vi "A Version Explorer - UI.vi"() -> ()   [LabVIEW 2020, in "A Version Explorer.lvlib"]
uses:
  A Version Explorer.lvlib
  Session/Session.lvclass
  <vilib>/Utility/miscctls.llb/LVRowAndColumnUnsignedTypeDef.ctl
  <vilib>/Utility/miscctls.llb/LVRowAndColumnTypeDef.ctl
  Session/Session.lvclass/Session.ctl
  <userlib>/_OpenG.lib/file/file.llb/Valid Path - Traditional__ogtk.vi
  <userlib>/_OpenG.lib/array/array.llb/Index 1D Array Elements (String)__ogtk.vi
panel:
  in  "Project Folder":path
  in  "Select All/Some/None":enum8{"False", "True", "Mixed"}(c332)
  in  "Refresh":bool
  in  "Save for Previous Version":bool
  in  "LabVIEW Version":string(combo)
  in  "Files":i32[](listbox)
  out "Status":string
  in  "OK":bool
  # "1) Select a Project Folder with files you wish to save to an earlier version of LabVIEW.\n    (Make note of the current LabVIEW version of each file using the listbox below.)"
  # "2) Select the project files in the listbox below that you\nwish to save to a different LabVIEW Version.\n\n(Ctrl+A selects all files, Ctrl+Click selects individual files.)"
  # "3) Select the target LabVIEW version.\n4) Press \"Save Selected Files\""
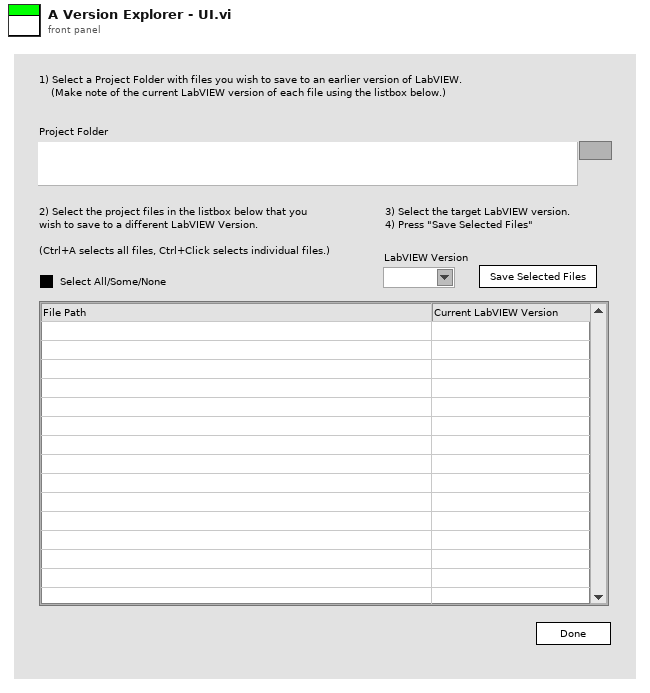
[diagram p1: front panel]
types:
  T1 = enum32{"Invalid", "Standard", "Closed", "Hidden", "Minimized", "Maximized"}
  T2 = enum32{"invalid app kind", "Development System", "Run Time System", "Student Edition", "Embedded LabVIEW", "Evaluation", "Custom"}
  T3 = typedef "LVRowAndColumnUnsignedTypeDef.ctl" = cluster{"Row":u32, "Column":u32}
  T4 = typedef "LVRowAndColumnTypeDef.ctl" = cluster{"Row":i32, "Column":i32}
  T5 = typedef "eventvkey.ctl" = enum16{"ASCII", "Enter", "Return", "Shift", "Ctrl", "Alt", "Cmd", "Opt", "Caps", "NumLock", "Clear", "Break", "Up", "Down", "Left", "Right", "Insert", "Delete", "Home", "End", "PageUp", "PageDown", "Escape", "Help", "Pause", "ScrollLock", "F1", "F2", "F3", "F4", "F5", "F6", "F7", "F8", "F9", "F10", "F11", "F12", "F13", "F14", "F15", "F16", "F17", "F18", "F19", "F20", "F21", "F22", "F23", "F24", "Play", "VolumeUp", "VolumeDown", "Mute", "Two Byte Char"}
  T6 = cluster{"Shift":bool, "Ctrl":bool, "Alt":bool, "Cmd":bool, "Opt":bool}
  T7 = cluster{"Core":cluster{"Current VI Reference":refnum<vi>, "Close Panel on Exit?":bool}, "Your Boolean data":bool, "Session":refnum<class "Session.lvclass">}
  T8 = cluster{"Current VI Reference":refnum<vi>, "Close Panel on Exit?":bool}
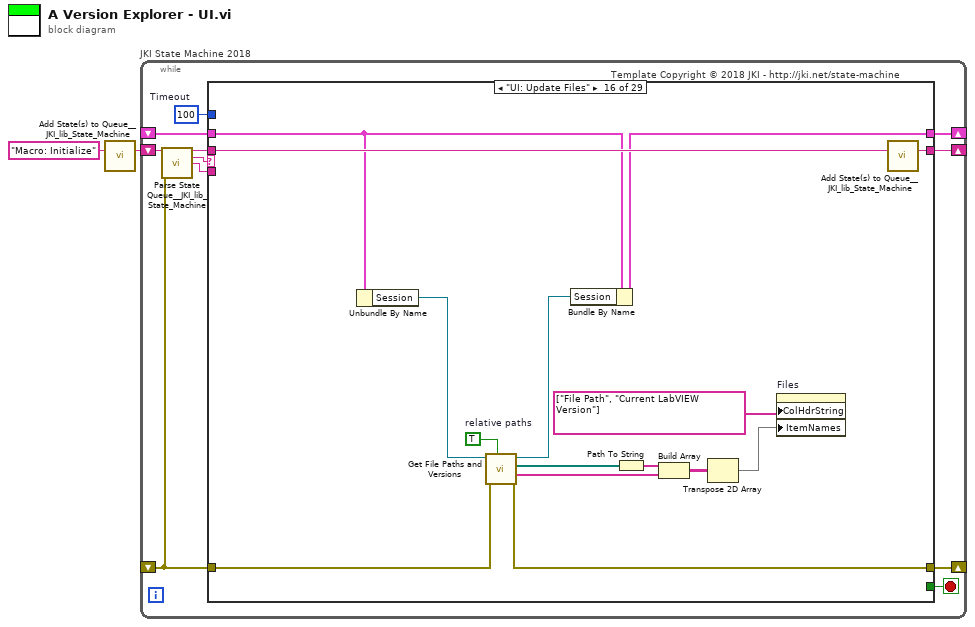
[diagram p0: block diagram]
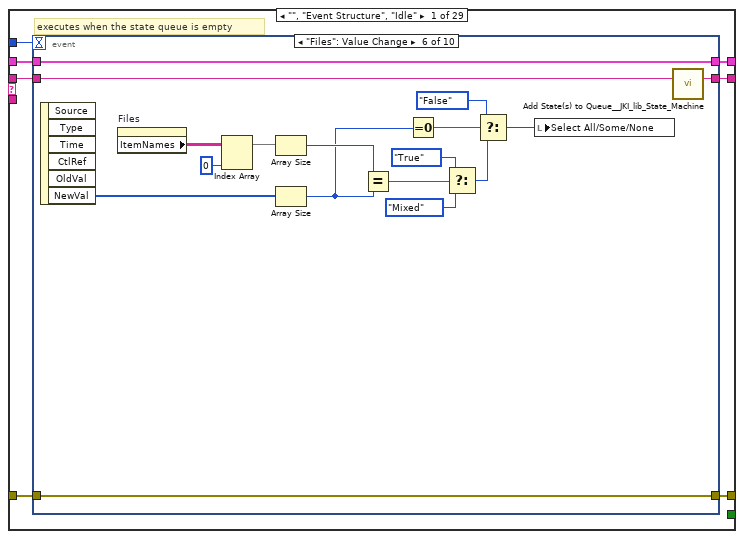
[diagram p2: hidden frame]
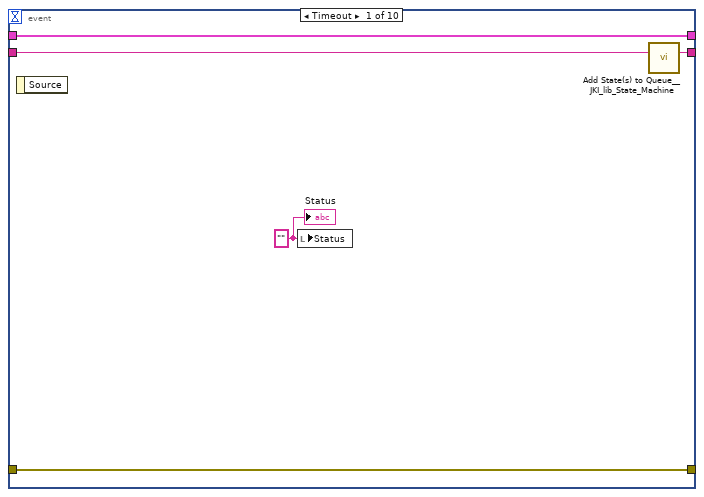
[diagram p3: hidden frame]
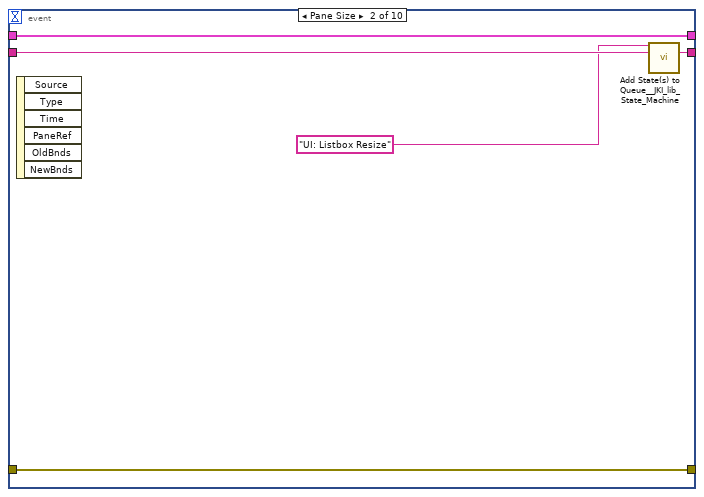
[diagram p4: hidden frame]
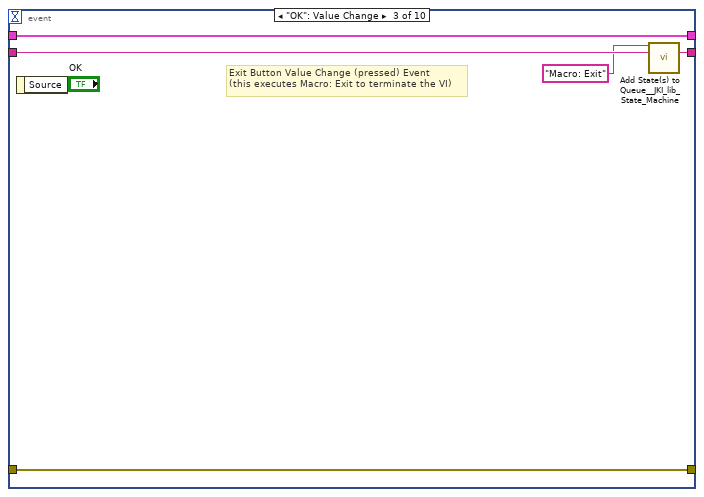
[diagram p5: hidden frame]
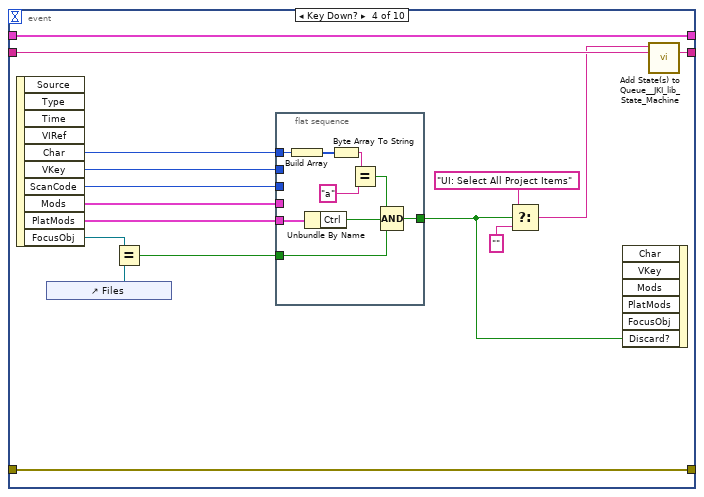
[diagram p6: hidden frame]
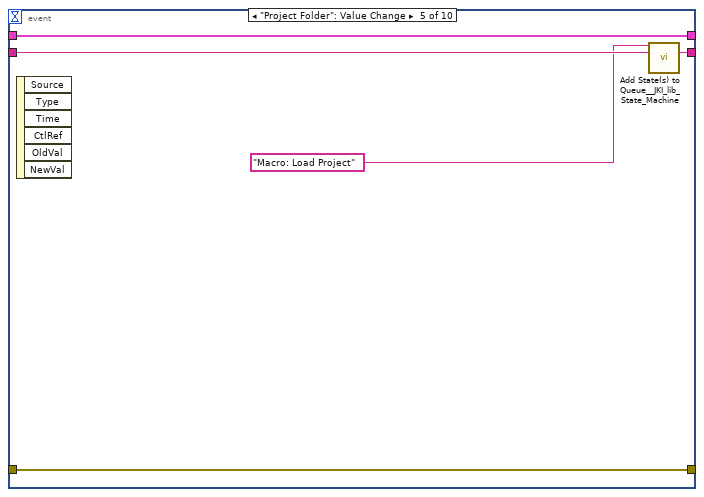
[diagram p7: hidden frame]
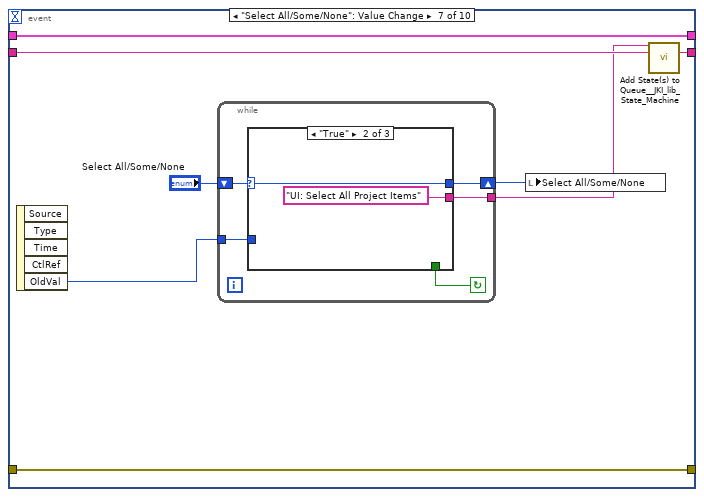
[diagram p8: hidden frame]
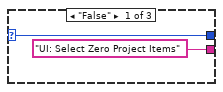
[diagram p9: hidden frame]
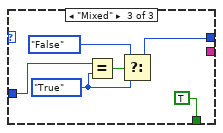
[diagram p10: hidden frame]
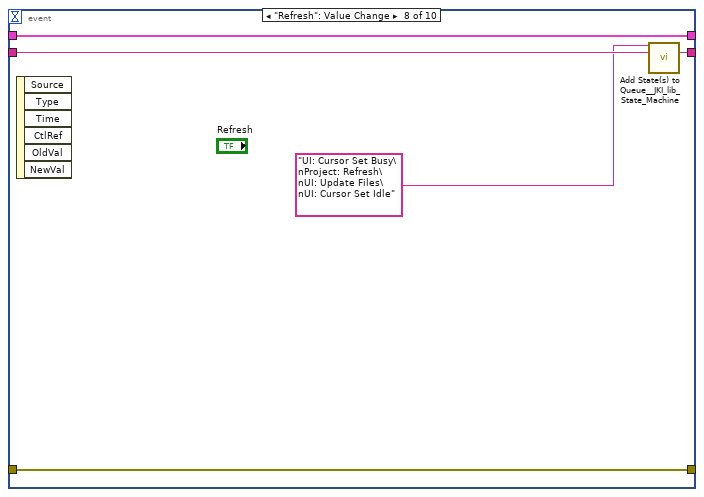
[diagram p11: hidden frame]
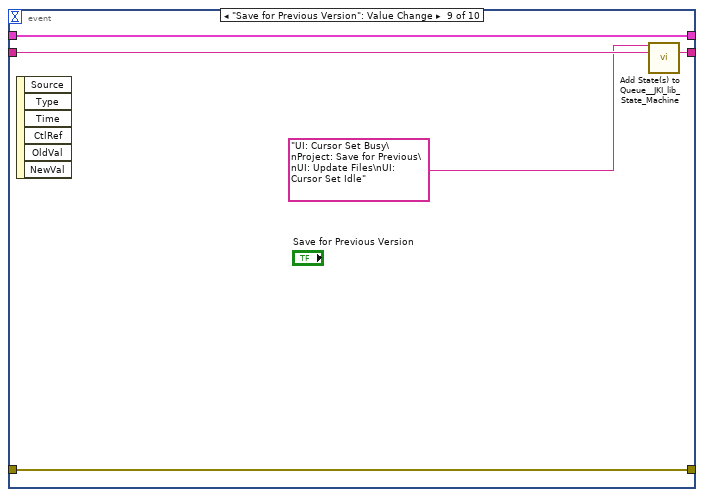
[diagram p12: hidden frame]
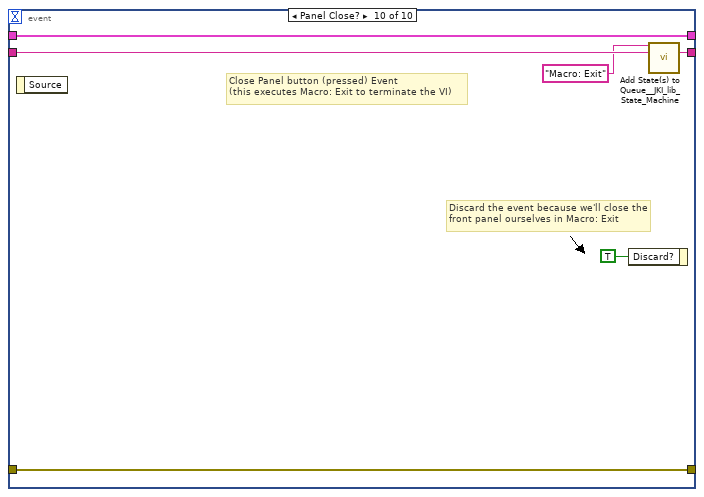
[diagram p13: hidden frame]
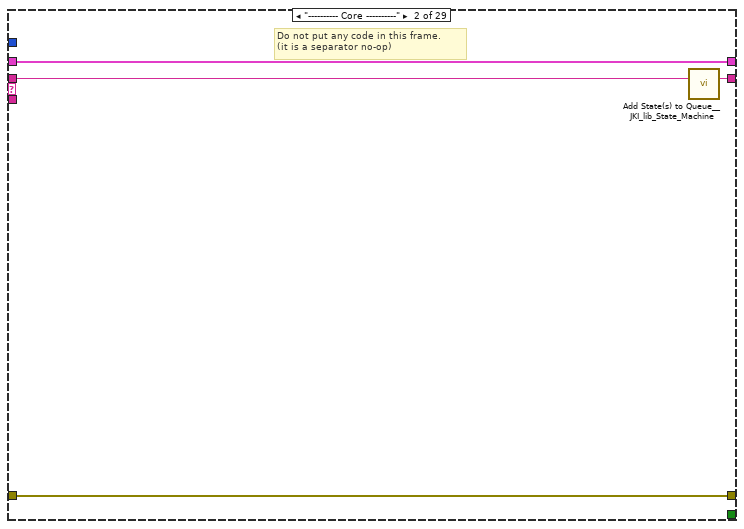
[diagram p14: hidden frame]
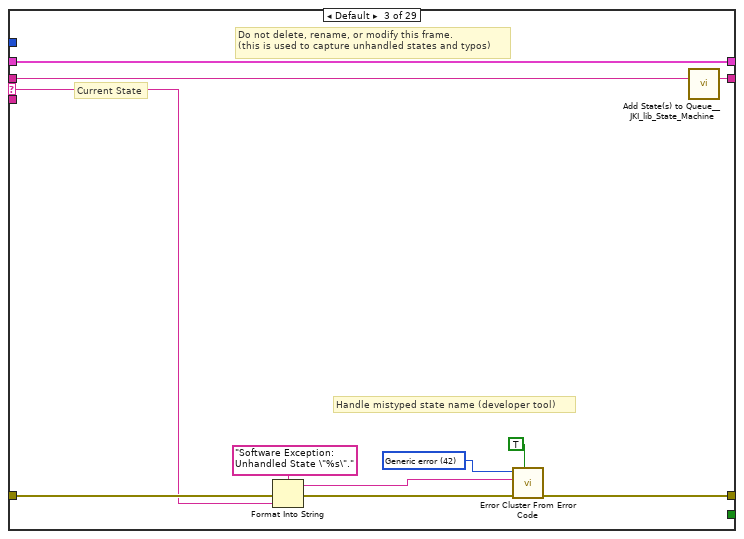
[diagram p15: hidden frame]
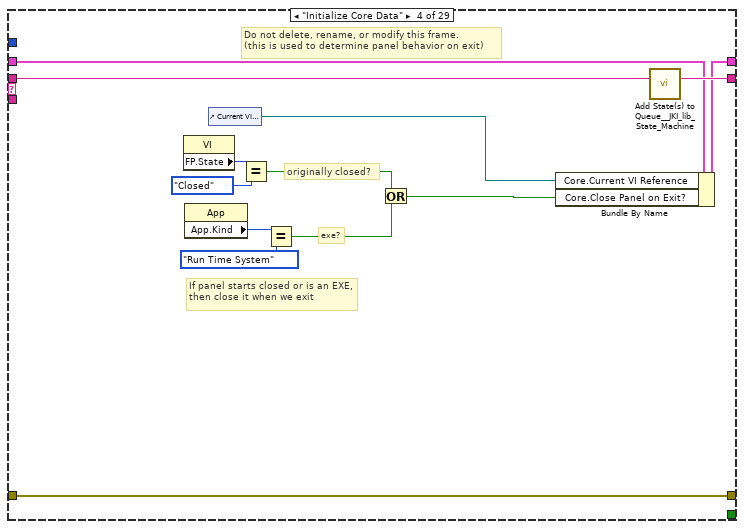
[diagram p16: hidden frame]
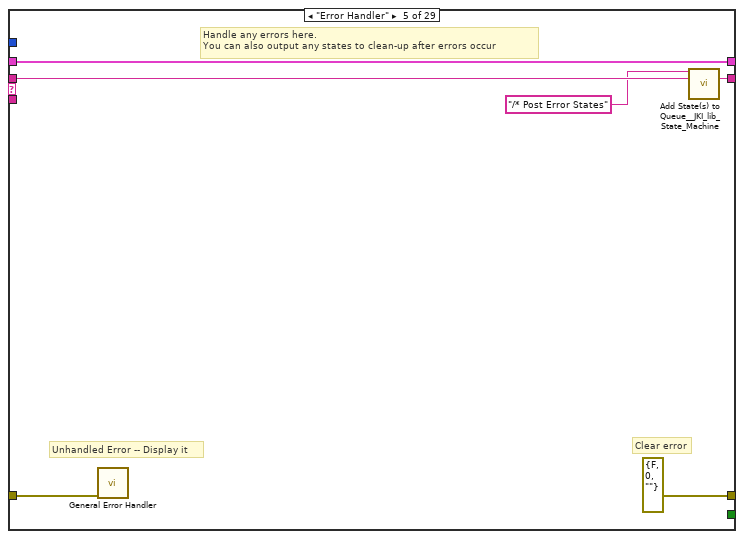
[diagram p17: hidden frame]
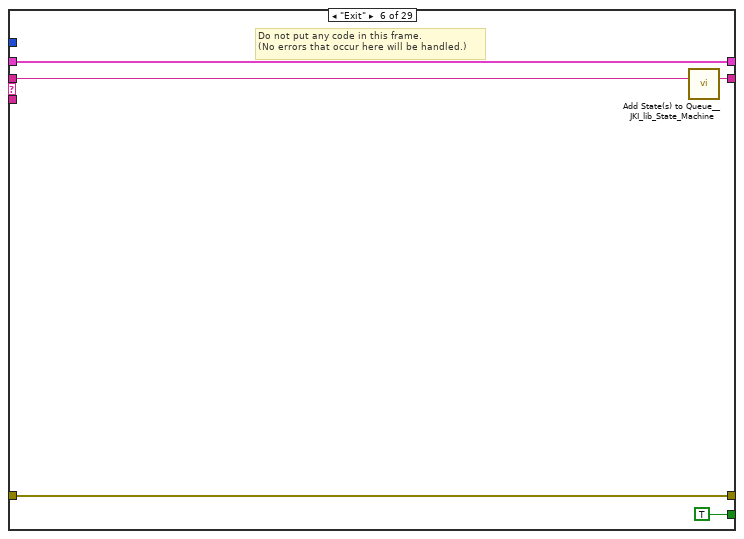
[diagram p18: hidden frame]
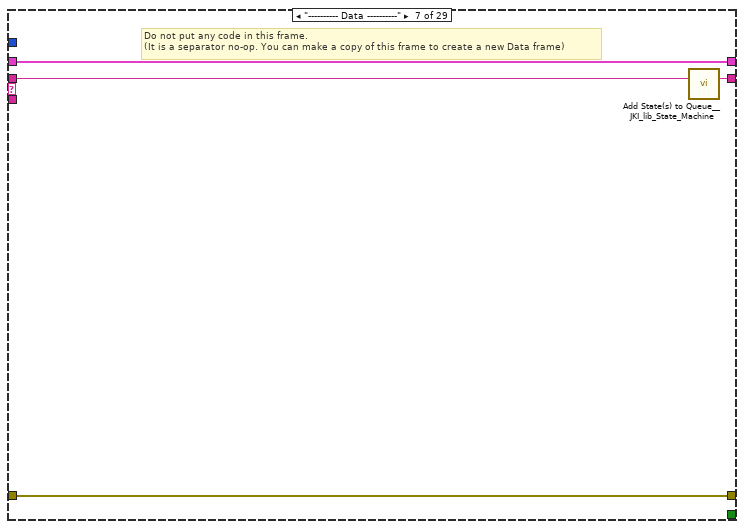
[diagram p19: hidden frame]
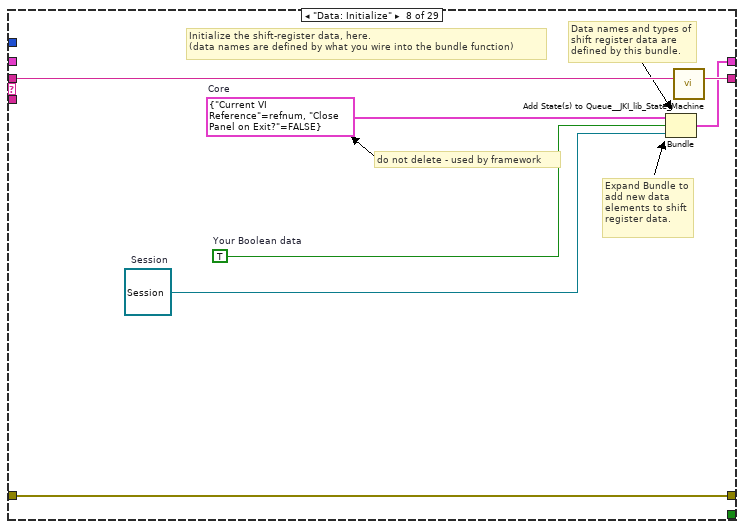
[diagram p20: hidden frame]
diagram:
  n1 = call <vilib>:"Add State(s) to Queue__JKI_lib_State_Machine.vi"("State(s) in (\"\")"="Macro: Initialize") -> ("States Out"=w2:string)  [unwired: 14 in]
  n2 = while "JKI State Machine 2018" {
    shift-right: [w6] -> _
    shift-left: _ -> [w5]
    shift-right: [w9] -> _
    shift-left: _ -> [w3]
    shift-right: [w8] -> _
    shift-left: w2 -> [w10]
    stop <- w7 stop-if-true
    w4 = 100  # Timeout
    # "Template Copyright © 2018 JKI - http://jki.net/state-machine"
    n3 = call <vilib>:"Parse State Queue__JKI_lib_State_Machine.vi"("State Queue"=w10, "Error In (no error)"=w3) -> ("Remaining States"=w12:string, "Current State"=w13:string, "Arguments"=w11:string)  [unwired: 11 in]
    n4 = case shown="\"UI: Update Files\"" w13 {
      selector: w13 -> [_ _ w126 _ _ _ _ _ _ _ _ _ _ _ _ _ _ _ _ _ _ _ _ _ _ _ _ _ _]
      tunnel: w12 -> [w20 w125 w130 w149 w155 w160 w164 w171 w177 w181 w185 w189 w196 w203 w208 w223 w228 w237 w247 w253 w264 w333 w343 w348 w358 w362 w373 w382 w401]
      tunnel: w11 -> [_ _ _ _ _ _ _ _ _ _ _ _ _ _ _ _ _ _ _ w248 w258 _ _ _ _ _ _ _ _]
      tunnel: w5 -> [w18 w122 w128 w142 w152 w158 w161 _ w172 w178 w182 w186 w193 w200 w205 w212 w226 w235 w245 w251 w260 w330 w340 w345 w355 w360 w371 w376 w398]
      tunnel: [w17 w123 w132 w146 errorcluster {"status"=FALSE, "code"=0, "source"=""} ("error out") w157 w162 w168 w173 w179 w183 w187 w194 w201 w206 w215 w225 w234 w244 w249 w261 w331 w341 w346 w356 w359 w367 w378 w399] -> w9
      tunnel: w3 -> [w16 w123 w131 w146 w151 w157 w162 w168 w174 w179 w183 w187 w194 w201 w206 w214 w225 w234 w244 w250 w262 w331 w341 w346 w356 w359 w366 w379 w386]
      tunnel: [w19 w124 w129 w148 w154 w159 w163 w170 w176 w180 w184 w188 w195 w202 w207 w222 w227 w236 w246 w252 w263 w332 w342 w347 w357 w361 w372 w381 w400] -> w8
      tunnel: [_ _ _ _ _ TRUE _ _ _ _ _ _ _ _ _ _ _ _ _ _ _ _ _ _ _ _ _ _ _] -> w7
      tunnel: [w15 w122 w128 w147 w152 w158 w161 w169 w172 w178 w182 w186 w193 w200 w205 w210 w226 w235 w245 w251 w260 w330 w340 w345 w355 w360 w365 w380 w397] -> w6
      tunnel: w4 -> [w14 _ _ _ _ _ _ _ _ _ _ _ _ _ _ _ _ _ _ _ _ _ _ _ _ _ _ _ _]
      frame "", "Event Structure", "Idle" {
        # "executes when the state queue is empty"
        n5 = event shown="[5] \"Files\": Value Change" {
          selector: _ -> [_ _ _ _ _ _ _ _ _ _]
          dyn-events: _ -> [_ _ _ _ _ _ _ _ _ _]
          timeout: w14 -> [_ _ _ _ _ _ _ _ _ _]
          tunnel: w20 -> [w25 w30 w35 w51 w65 w82 w90 w110 w115 w121]
          tunnel: [w24 w29 w34 w50 w64 w81 w89 w109 w114 w120] -> w19
          tunnel: w18 -> [w22 w27 w32 w48 w62 w79 w87 w107 w112 w118]
          tunnel: [w23 w28 w33 w49 w63 w80 w88 w108 w113 w119] -> w17
          tunnel: w16 -> [w23 w28 w33 w49 w63 w80 w88 w108 w113 w119]
          tunnel: [w22 w27 w32 w48 w62 w79 w87 w107 w112 w118] -> w15
          event Timeout {
            w21 = "" ("Status")
            n6 = event-data() -> ()  [unwired: 1 in, 1 out]
            n7 = local write "Status"(w21) -> ()
            n8 = call <vilib>:"Add State(s) to Queue__JKI_lib_State_Machine.vi"("State(s) in (\"\")"=w25) -> ("States Out"=w24:string)  [unwired: 14 in]
            "Status" <- w21
          }
          event Pane Size {
            n9 = event-data() -> ()  [unwired: 1 in, 6 out]
            n10 = call <vilib>:"Add State(s) to Queue__JKI_lib_State_Machine.vi"("State(s) in Front (\"\")"="UI: Listbox Resize" ("Status"), "State(s) in (\"\")"=w30) -> ("States Out"=w29:string)  [unwired: 13 in]
          }
          event "OK": Value Change {
            # "Exit Button Value Change (pressed) Event\n(this executes Macro: Exit to terminate the VI)"
            n11 = event-data() -> ()  [unwired: 1 in, 1 out]
            n12 = call <vilib>:"Add State(s) to Queue__JKI_lib_State_Machine.vi"("State(s) in Front (\"\")"="Macro: Exit", "State(s) in (\"\")"=w35) -> ("States Out"=w34:string)  [unwired: 13 in]
          }
          event Key Down? {
            n13 = event-data() -> ("Char"=w41:i16, "VKey"=w42:T5, "ScanCode"=w43:i16, "Mods"=w47:cluster{"Num Pad":bool, "Menu Key":bool}, "PlatMods"=w46:T6, "FocusObj"=w45:refnum<vi>)  [unwired: 1 in, 4 out]
            n14 = control-ref of="Files"() -> (w44:refnum<vi>)
            n15 = Equal?(x=w45, y=w44) -> (x = y?=w40:bool)
            n16 = flat-sequence {
              tunnel: w47 -> [_]
              tunnel: w46 -> [w60]
              tunnel: w43 -> [_]
              tunnel: w42 -> [_]
              tunnel: w41 -> [w59]
              tunnel: w40 -> [w53]
              tunnel: [w52] -> w39
              frame #0 {
                n17 = Build Array(w59) -> (w58:i16[])
                n18 = Unbundle By Name(w60) -> ("Ctrl"=w54:bool)
                n19 = Byte Array To String(unsigned byte array=w58) -> (string=w57:string)
                n20 = Equal?(x=w57, y="a" ("string")) -> (x = y?=w55:bool)
                n21 = Compound Arithmetic op=AND(w55, w54, w53) -> (w52:bool)
              }
            }
            n22 = Select(t="UI: Select All Project Items", s=w39, f="") -> (s? t:f=w36:string)
            n23 = event-data("Discard?"=w39) -> ()  [unwired: 6 in, 1 out]
            n24 = call <vilib>:"Add State(s) to Queue__JKI_lib_State_Machine.vi"("State(s) in Front (\"\")"=w36, "State(s) in (\"\")"=w51) -> ("States Out"=w50:string)  [unwired: 13 in]
          }
          event "Project Folder": Value Change {
            n25 = event-data() -> ()  [unwired: 1 in, 6 out]
            n26 = call <vilib>:"Add State(s) to Queue__JKI_lib_State_Machine.vi"("State(s) in Front (\"\")"="Macro: Load Project", "State(s) in (\"\")"=w65) -> ("States Out"=w64:string)  [unwired: 13 in]
          }
          event "Files": Value Change {
            n27 = event-data() -> ("NewVal"=w77:i32[])  [unwired: 1 in, 5 out]
            n28 = property on="Files" class="MCListbox (strict)"() -> ("ItemNames"=w78:string[][])  [unwired: 2 in, 2 out]
            n29 = Index Array(array=w78, index (col)=0 ("disabled index (col)")) -> (element=w75:string[])  [unwired: 1 in]
            n30 = Array Size(array=w75) -> (size(s)=w76:i32)
            n31 = Array Size(array=w77) -> (size(s)=w73:i32)
            n32 = Equal?(x=w76, y=w73) -> (x = y?=w69:bool)
            n33 = Equal To 0?(x=w73) -> (x = 0?=w72:bool)
            n34 = Select(t=enum8{"False", "True", "Mixed"}."True" ("Select All/Some/None"), s=w69, f=enum8{"False", "True", "Mixed"}."Mixed" ("Select All/Some/None")) -> (s? t:f=w66:enum8{"False", "True", "Mixed"})
            n35 = Select(t=enum8{"False", "True", "Mixed"}."False" ("Select All/Some/None"), s=w72, f=w66) -> (s? t:f=w70:enum8{"False", "True", "Mixed"})
            n36 = local write "Select All/Some/None"(w70) -> ()
            n37 = call <vilib>:"Add State(s) to Queue__JKI_lib_State_Machine.vi"("State(s) in (\"\")"=w82) -> ("States Out"=w81:string)  [unwired: 14 in]
          }
          event "Select All/Some/None": Value Change {
            n38 = event-data() -> ("OldVal"=w84:enum8{"False", "True", "Mixed"})  [unwired: 1 in, 4 out]
            n39 = while {
              tunnel: [w94] -> w85
              tunnel: w84 -> [w93]
              shift-right: [w91] -> w83
              shift-left: "Select All/Some/None" -> [w95]
              stop <- w92 continue-if-true
              n40 = case shown="\"True\"" w95 {
                selector: w95 -> [w96 w98 _]
                tunnel: ["UI: Select Zero Project Items" "UI: Select All Project Items" _] -> w94
                tunnel: w93 -> [_ _ w104]
                tunnel: [_ _ TRUE] -> w92
                tunnel: [w96 w98 w100] -> w91
                frame "False" {
                }
                frame "True" {
                }
                frame "Mixed" {
                  w102 = enum8{"False", "True", "Mixed"}."True" ("Select All/Some/None")
                  n41 = Equal?(x=w104, y=w102) -> (x = y?=w103:bool)
                  n42 = Select(t=enum8{"False", "True", "Mixed"}."False" ("Select All/Some/None"), s=w103, f=w102) -> (s? t:f=w100:enum8{"False", "True", "Mixed"})
                }
              }
            }
            n43 = local write "Select All/Some/None"(w83) -> ()
            n44 = call <vilib>:"Add State(s) to Queue__JKI_lib_State_Machine.vi"("State(s) in Front (\"\")"=w85, "State(s) in (\"\")"=w90) -> ("States Out"=w89:string)  [unwired: 13 in]
          }
          event "Refresh": Value Change {
            n45 = event-data() -> ()  [unwired: 1 in, 6 out]
            n46 = call <vilib>:"Add State(s) to Queue__JKI_lib_State_Machine.vi"("State(s) in Front (\"\")"="UI: Cursor Set Busy\nProject: Refresh\nUI: Update Files\nUI: Cursor Set Idle", "State(s) in (\"\")"=w110) -> ("States Out"=w109:string)  [unwired: 13 in]
          }
          event "Save for Previous Version": Value Change {
            n47 = event-data() -> ()  [unwired: 1 in, 6 out]
            n48 = call <vilib>:"Add State(s) to Queue__JKI_lib_State_Machine.vi"("State(s) in Front (\"\")"="UI: Cursor Set Busy\nProject: Save for Previous\nUI: Update Files\nUI: Cursor Set Idle", "State(s) in (\"\")"=w115) -> ("States Out"=w114:string)  [unwired: 13 in]
          }
          event Panel Close? {
            # "Discard the event because we'll close the front panel ourselves in Macro: Exit"
            # "Close Panel button (pressed) Event\n(this executes Macro: Exit to terminate the VI)"
            n49 = event-data() -> ()  [unwired: 1 in, 1 out]
            n50 = event-data("Discard?"=TRUE) -> ()  [unwired: 1 in, 1 out]
            n51 = call <vilib>:"Add State(s) to Queue__JKI_lib_State_Machine.vi"("State(s) in Front (\"\")"="Macro: Exit", "State(s) in (\"\")"=w121) -> ("States Out"=w120:string)  [unwired: 13 in]
          }
        }
      }
      frame "---------- Core ----------" {
        # "Do not put any code in this frame.\n(it is a separator no-op)"
        n52 = call <vilib>:"Add State(s) to Queue__JKI_lib_State_Machine.vi"("State(s) in (\"\")"=w125) -> ("States Out"=w124:string)  [unwired: 14 in]
      }
      frame Default {
        w135 = 42 items=["No error", "Argument error", "Memory is full", "Out of zone", "End of file", "File already open", "Generic file I/O error", "File not found", "File permission error", "Disk is full", "Duplicate path", "Too many files open", "System feature not enabled", "Resource file not found", "Cannot add resource", "Resource not found", "Image not found", "Image memory error", "Pen does not exist", "Config type invalid", "Config token not found", "Config parse error", "Config memory error", "Bad external code format", "Bad external code offset", "External code not present", "Null window", "Destroy window error", "Null menu", "Print aborted", "Bad print record", "Print driver error", "Windows error during printing", "Memory error during printing", "Print dialog error", "Generic print error", "Invalid device refnum", "Device not found", "Device parameter error", "Device unit error", "Cannot open device", "Device call aborted", "Generic error", "Cancelled by user", "Object ID too low", "Object ID too high", "Object not in heap", "Unknown heap", "Unknown object (invalid DefProc)", "Unknown object (DefProc not in table)", "Message out of range", "Invalid (null) method", "Unknown message", "Manager call not supported", "Bad address", "Network operation in progress", "Network operation timed out", "Connection is busy", "Network attribute not supported", "Network error", "Address in use", "System out of memory", "Connection aborted", "Connection refused", "Not connected", "Already connected", "Connection closed", "Initialization error (interapplication manager)", "Bad occurrence", "Wait on unbound occurrence handler", "Occurrence queue overflow", "Datalog type conflict", "Unused", "Unrecognized type (interapplication manager)", "Memory corrupt", "Failed to make temporary DLL", "Old CIN version", "Drag socket not found", "Failed to load drop-object", "Failed to register OLE object", "Failed to release OLE object", "Format specifier type mismatch", "Unknown format specifier", "Too few format specifiers", "Too many format specifiers", "Scan failed", "Newer CIN version", "Error converting to variant", "Runtime menu error", "Password tampered", "Variant attribute not found", "Incompatible variant data type", "Event data is not available", "Event Store is not present", "Occurrence is not found", "Event Queue is not created", "Event info is not available", "Refnum passed is NULL", "Error retrieving Class GUID", "Error retrieving CoClass GUID", "Error retrieving TypeLib GUID.", "Bad built application magic bytes.", "Specific driver is different from the specific driver associated with the Logical Name.", "There is no session opened to the class driver.", "Max Error", "MAX - Error with config objects", "MAX - Error loading configuration", "MAX - Group not supported"]
        # "Current State"
        # "Do not delete, rename, or modify this frame.\n(this is used to capture unhandled states and typos)"
        # "Handle mistyped state name (developer tool)"
        n53 = Format Into String(format string="Software Exception: Unhandled State \"%s\"." ("message"), error in=w131, w126) -> (resulting string=w134:string, error out=w133:errorcluster)  [unwired: 1 in]
        n54 = call <vilib>:"Error Cluster From Error Code.vi"("show call chain? (False)"=TRUE, "error in (no error)"=w133, "error message (\"\")"=w134, "error code (0)"=w135) -> ("error out"=w132:errorcluster)  [unwired: 5 in]
        n55 = call <vilib>:"Add State(s) to Queue__JKI_lib_State_Machine.vi"("State(s) in (\"\")"=w130) -> ("States Out"=w129:string)  [unwired: 14 in]
      }
      frame "Initialize Core Data" {
        # "Do not delete, rename, or modify this frame.\n(this is used to determine panel behavior on exit)"
        # "originally closed?"
        # "exe?"
        # "If panel starts closed or is an EXE, then close it when we exit"
        n56 = property class="VI"() -> ("FP.State"=w139:T1)  [unwired: 2 in, 2 out]
        n57 = property class="App"() -> ("App.Kind"=w145:T2)  [unwired: 2 in, 2 out]
        n58 = control-ref of="Current VI Reference"() -> (w140:refnum<vi>)
        n59 = Equal?(x=w139, y=T1."Closed" ("Front Panel Window:State")) -> (x = y?=w137:bool)
        n60 = Equal?(x=w145, y=T2."Run Time System" ("Application:Kind")) -> (x = y?=w143:bool)
        n61 = Or(x=w137, y=w143) -> (x .or. y?=w141:bool)
        n62 = Bundle By Name(cluster=w142, "Core.Current VI Reference"=w140, "Core.Close Panel on Exit?"=w141) -> (w147:T7)
        n63 = call <vilib>:"Add State(s) to Queue__JKI_lib_State_Machine.vi"("State(s) in (\"\")"=w149) -> ("States Out"=w148:string)  [unwired: 14 in]
      }
      frame "Error Handler" {
        # "Unhandled Error -- Display it"
        # "Handle any errors here.\nYou can also output any states to clean-up after errors occur"
        # "Clear error"
        n64 = call <vilib>:"General Error Handler.vi"("error in (no error)"=w151) -> ()  [unwired: 10 in, 5 out]
        n65 = call <vilib>:"Add State(s) to Queue__JKI_lib_State_Machine.vi"("State(s) in Front (\"\")"="/* Post Error States", "State(s) in (\"\")"=w155) -> ("States Out"=w154:string)  [unwired: 13 in]
      }
      frame "Exit" {
        # "Do not put any code in this frame.\n(No errors that occur here will be handled.)"
        n66 = call <vilib>:"Add State(s) to Queue__JKI_lib_State_Machine.vi"("State(s) in (\"\")"=w160) -> ("States Out"=w159:string)  [unwired: 14 in]
      }
      frame "---------- Data ----------" {
        # "Do not put any code in this frame.\n(It is a separator no-op. You can make a copy of this frame to create a new Data frame)"
        n67 = call <vilib>:"Add State(s) to Queue__JKI_lib_State_Machine.vi"("State(s) in (\"\")"=w164) -> ("States Out"=w163:string)  [unwired: 14 in]
      }
      frame "Data: Initialize" {
        w165 = refnum<class "Session.lvclass"> refnum  # Session
        w166 = T8 {"Current VI Reference"=refnum, "Close Panel on Exit?"=FALSE}  # Core
        w167 = TRUE  # Your Boolean data
        # "do not delete - used by framework"
        # "Expand Bundle to add new data elements to shift register data."
        # "Data names and types of shift register data are defined by this bundle."
        # "Initialize the shift-register data, here.\n(data names are defined by what you wire into the bundle function)"
        n68 = Bundle("Core"=w166, "Your Boolean data"=w167, "Session"=w165) -> (w169:T7)  [unwired: 1 in]
        n69 = call <vilib>:"Add State(s) to Queue__JKI_lib_State_Machine.vi"("State(s) in (\"\")"=w171) -> ("States Out"=w170:string)  [unwired: 14 in]
      }
      frame "Data: Cleanup" {
        # "Cleanup any data and references, here.\n(this is called automatically, by the Macro: Exit)"
        n70 = Unbundle By Name(w172) -> ("Core.Current VI Reference"=w175:refnum<vi>)
        n71 = Close Reference(reference=w175, error in (no error)=w174) -> (error out=w173:errorcluster)
        n72 = call <vilib>:"Add State(s) to Queue__JKI_lib_State_Machine.vi"("State(s) in (\"\")"=w177) -> ("States Out"=w176:string)  [unwired: 14 in]
      }
      frame "---------- UI ----------" {
        # "Do not put any code in this frame.\n(It is a separator no-op. You can make a copy of this frame to create a new UI frame)"
        n73 = call <vilib>:"Add State(s) to Queue__JKI_lib_State_Machine.vi"("State(s) in (\"\")"=w181) -> ("States Out"=w180:string)  [unwired: 14 in]
      }
      frame "UI: Cursor Set Busy" {
        # "Do not put any code in this frame.\n(It is a separator no-op. You can make a copy of this frame to create a new UI frame)"
        n74 = call <vilib>:"Set Busy.vi"() -> ()  [unwired: 10 in, 2 out]
        n75 = call <vilib>:"Add State(s) to Queue__JKI_lib_State_Machine.vi"("State(s) in (\"\")"=w185) -> ("States Out"=w184:string)  [unwired: 14 in]
      }
      frame "UI: Cursor Set Idle" {
        # "Do not put any code in this frame.\n(It is a separator no-op. You can make a copy of this frame to create a new UI frame)"
        n76 = call <vilib>:"Unset Busy.vi"() -> ()  [unwired: 11 in, 1 out]
        n77 = call <vilib>:"Add State(s) to Queue__JKI_lib_State_Machine.vi"("State(s) in (\"\")"=w189) -> ("States Out"=w188:string)  [unwired: 14 in]
      }
      frame "UI: Select All Project Items" {
        # "Do not put any code in this frame.\n(It is a separator no-op. You can make a copy of this frame to create a new UI frame)"
        n78 = property on="Files" class="MCListbox (strict)"() -> ("ItemNames"=w192:string[][])  [unwired: 2 in, 2 out]
        n79 = local write "Select All/Some/None"(enum8{"False", "True", "Mixed"}."True" ("Select All/Some/None")) -> ()
        n80 = for {
          tunnel: w192 -> [_] mode=indexing
          tunnel: [w197] -> w191 mode=indexing
          i -> [w197]
        }
        n81 = property on="Files" class="MCListbox (strict)"("Value"=w191) -> ()  [unwired: 2 in, 2 out]
        n82 = call <vilib>:"Add State(s) to Queue__JKI_lib_State_Machine.vi"("State(s) in (\"\")"=w196) -> ("States Out"=w195:string)  [unwired: 14 in]
      }
      frame "UI: Select Zero Project Items" {
        n83 = local write "Select All/Some/None"(enum8{"False", "True", "Mixed"}."False" ("Select All/Some/None")) -> ()
        n84 = property on="Files" class="MCListbox (strict)"("Value"=i32[] [] ("Files")) -> ()  [unwired: 2 in, 2 out]
        n85 = call <vilib>:"Add State(s) to Queue__JKI_lib_State_Machine.vi"("State(s) in (\"\")"=w203) -> ("States Out"=w202:string)  [unwired: 14 in]
      }
      frame "UI: Show First Row of Project Items" {
        n86 = property on="Files" class="MCListbox (strict)"("TopLeft"=T3 {"Row"=0, "Column"=0} ("Top Left Visible Cell")) -> ()  [unwired: 2 in, 2 out]
        n87 = call <vilib>:"Add State(s) to Queue__JKI_lib_State_Machine.vi"("State(s) in (\"\")"=w208) -> ("States Out"=w207:string)  [unwired: 14 in]
      }
      frame "UI: Update Files" {
        w216 = TRUE  # relative paths
        n88 = Unbundle By Name(w212) -> ("Session"=w211:refnum<class "Session.lvclass">)
        n89 = call "Get File Paths and Versions.vi"("relative paths? (F: Absolute)"=w216, "error in (no error)"=w214, "Session in"=w211) -> ("error out"=w215:errorcluster, "Versions"=w218:string[], "File Paths"=w220:path[], "Session out"=w209:refnum<class "Session.lvclass">)  [unwired: 5 in]
        n90 = Bundle By Name(cluster=w212, "Session"=w209) -> (w210:T7)
        n91 = Path To String(path=w220) -> (string=w219:string[])
        n92 = Build Array(w219, w218) -> (w217:string[][])
        n93 = Transpose 2D Array(2D array=w217) -> (transposed array=w213:string[][])
        n94 = property on="Files" class="MCListbox (strict)"("ColHdrString"=string[] ["File Path", "Current LabVIEW Version"] ("Row Header Strings[]"), "ItemNames"=w213) -> ()  [unwired: 2 in, 2 out]
        n95 = call <vilib>:"Add State(s) to Queue__JKI_lib_State_Machine.vi"("State(s) in (\"\")"=w223) -> ("States Out"=w222:string)  [unwired: 14 in]
      }
      frame "UI: Initialize" {
        # "Initialize the User Interface, here.\n(this is called automatically, by the Macro: Init)"
        n96 = local write "Status"("" ("Status")) -> ()
        n97 = call <vilib>:"Add State(s) to Queue__JKI_lib_State_Machine.vi"("State(s) in (\"\")"=w228) -> ("States Out"=w227:string)  [unwired: 14 in]
      }
      frame "UI: Uninitialize" {
        n98 = property class="App"() -> ("App.Version"=w230:string)  [unwired: 2 in, 2 out]
        n99 = Match Pattern(string=w230, regular expression="[0-9]+\\.[0-9]+") -> (match substring=w229:string)  [unwired: 1 in, 3 out]
        n100 = local write "LabVIEW Version"(w229) -> ()
        n101 = local write "Status"("" ("Status")) -> ()
        n102 = property on="Files" class="MCListbox (strict)"("ItemNames"=string[][] [] ("Item Names")) -> ()  [unwired: 2 in, 2 out]
        n103 = call <vilib>:"Add State(s) to Queue__JKI_lib_State_Machine.vi"("State(s) in (\"\")"=w237) -> ("States Out"=w236:string)  [unwired: 14 in]
      }
      frame "UI: Listbox Resize" {
        w239 = 160 ("y")
        n104 = property on="Files" class="MCListbox (strict)"() -> ("ContentRectBoundsWidth"=w241:i32)  [unwired: 2 in, 2 out]
        n105 = Subtract(x=w241, y=w239) -> (x-y=w242:i32)
        n106 = property on="Files" class="MCListbox (strict)"("ActiveCell"=T4 {"Row"=-2, "Column"=0} ("Active Cell:Active Cell"), "Width"=w242) -> (error out=w243:errorcluster)  [unwired: 2 in, 1 out]
        n107 = property on="Files" class="MCListbox (strict)"(error in=w243, "ActiveCell"=T4 {"Row"=-2, "Column"=1} ("Active Cell:Active Cell"), "Width"=w239) -> ()  [unwired: 1 in, 2 out]
        n108 = call <vilib>:"Add State(s) to Queue__JKI_lib_State_Machine.vi"("State(s) in (\"\")"=w247) -> ("States Out"=w246:string)  [unwired: 14 in]
      }
      frame "UI: Cursor Set" {
        # "Argument"
        # "Set and Unset Cursor Busy.\n(Usage: \"UI: Cursor Set >> Busy|Idle\")"
        n109 = case shown="\"Idle\", Default" w248 {
          tunnel: w250 -> [w255 w257]
          tunnel: [w254 w256] -> w249
          frame "Idle", Default {
            n110 = call <vilib>:"Unset Busy.vi"("error in (no error)"=w255) -> ("error out"=w254:errorcluster)  [unwired: 10 in]
          }
          frame "Busy" {
            n111 = call <vilib>:"Set Busy.vi"("error in (no error)"=w257) -> ("error out"=w256:errorcluster)  [unwired: 9 in, 1 out]
          }
        }
        n112 = call <vilib>:"Add State(s) to Queue__JKI_lib_State_Machine.vi"("State(s) in (\"\")"=w253) -> ("States Out"=w252:string)  [unwired: 14 in]
      }
      frame "UI: Front Panel State" {
        # "Argument"
        # "Set Front Panel Open or Closed\n(Usage: \"UI: Front Panel State >> Open|Close\")"
        n113 = Unbundle By Name(w260) -> ("Core.Current VI Reference"=w259:refnum<vi>)
        n114 = case shown="\"Minimize\", \"Minimized\"" w258 {
          tunnel: w262 -> [w270 w285 w296 w309 w322]
          tunnel: [w272 w286 w298 w311 w324] -> w261
          tunnel: w259 -> [w271 w283 w297 w310 w323]
          frame "Open", "Standard", Default {
            w265 = T1."Standard" ("State")
            n115 = property class="VI"(reference=w271, error in=w270) -> (reference out=w268:refnum<vi>, error out=w269:errorcluster, "FP.State"=w267:T1)
            n116 = Not Equal?(x=w267, y=w265) -> (x != y?=w266:bool)
            n117 = case shown="True" w266 {
              tunnel: [w276 w278] -> w272
              tunnel: w269 -> [w275 w278]
              tunnel: w268 -> [w274 _]
              tunnel: w265 -> [w273 _]
              frame True {
                n118 = invoke class="VI" method="FP.Open"(reference=w274, error in=w275, "Activate"=TRUE, "State"=w273) -> (error out=w276:errorcluster)  [unwired: 1 in, 4 out]
              }
              frame False {
              }
            }
          }
          frame "Close", "Closed" {
            n119 = property class="VI"(reference=w283, error in=w285) -> (reference out=w282:refnum<vi>, error out=w284:errorcluster, "FP.State"=w280:T1)
            n120 = Not Equal?(x=w280, y=T1."Closed" ("Front Panel Window:State")) -> (x != y?=w279:bool)
            n121 = case shown="True" w279 {
              tunnel: [w287 w290] -> w286
              tunnel: w284 -> [w287 w289]
              tunnel: w282 -> [_ w288]
              frame False {
              }
              frame True {
                n122 = invoke class="VI" method="FP.Close"(reference=w288, error in=w289) -> (error out=w290:errorcluster)  [unwired: 1 in, 2 out]
              }
            }
          }
          frame "Hidden", "Hide" {
            w291 = T1."Hidden" ("State")
            n123 = property class="VI"(reference=w297, error in=w296) -> (reference out=w294:refnum<vi>, error out=w295:errorcluster, "FP.State"=w293:T1)
            n124 = Not Equal?(x=w293, y=w291) -> (x != y?=w292:bool)
            n125 = case shown="True" w292 {
              tunnel: [w302 w303] -> w298
              tunnel: w295 -> [w301 w303]
              tunnel: w294 -> [w300 _]
              tunnel: w291 -> [w299 _]
              frame True {
                n126 = invoke class="VI" method="FP.Open"(reference=w300, error in=w301, "State"=w299) -> (error out=w302:errorcluster)  [unwired: 2 in, 4 out]
              }
              frame False {
              }
            }
          }
          frame "Minimize", "Minimized" {
            w304 = T1."Minimized" ("State")
            n127 = property class="VI"(reference=w310, error in=w309) -> (reference out=w307:refnum<vi>, error out=w308:errorcluster, "FP.State"=w306:T1)
            n128 = Not Equal?(x=w306, y=w304) -> (x != y?=w305:bool)
            n129 = case shown="True" w305 {
              tunnel: [w315 w316] -> w311
              tunnel: w308 -> [w314 w316]
              tunnel: w307 -> [w313 _]
              tunnel: w304 -> [w312 _]
              frame True {
                n130 = invoke class="VI" method="FP.Open"(reference=w313, error in=w314, "State"=w312) -> (error out=w315:errorcluster)  [unwired: 2 in, 4 out]
              }
              frame False {
              }
            }
          }
          frame "Maximize", "Maximized" {
            w317 = T1."Maximized" ("State")
            n131 = property class="VI"(reference=w323, error in=w322) -> (reference out=w320:refnum<vi>, error out=w321:errorcluster, "FP.State"=w319:T1)
            n132 = Not Equal?(x=w319, y=w317) -> (x != y?=w318:bool)
            n133 = case shown="True" w318 {
              tunnel: [w328 w329] -> w324
              tunnel: w321 -> [w327 w329]
              tunnel: w320 -> [w326 _]
              tunnel: w317 -> [w325 _]
              frame True {
                n134 = invoke class="VI" method="FP.Open"(reference=w326, error in=w327, "State"=w325) -> (error out=w328:errorcluster)  [unwired: 2 in, 4 out]
              }
              frame False {
              }
            }
          }
        }
        n135 = call <vilib>:"Add State(s) to Queue__JKI_lib_State_Machine.vi"("State(s) in (\"\")"=w264) -> ("States Out"=w263:string)  [unwired: 14 in]
      }
      frame "---------- Macro ----------" {
        # "Do not put any code in this frame.\n(It is a separator no-op. You can make a copy of this frame to create a new Macro frame)"
        n136 = call <vilib>:"Add State(s) to Queue__JKI_lib_State_Machine.vi"("State(s) in (\"\")"=w333) -> ("States Out"=w332:string)  [unwired: 14 in]
      }
      frame "Macro: Initialize" {
        w339 = "Data: Initialize\nInitialize Core Data\nUI: Initialize\nUI: Select Zero Project Items\nUI: Listbox Resize\nUI: Front Panel State >> Open"  # Data: Initialize Initialize Core Data UI: Initialize UI: Select Zero Project Items UI: Listbox Resize UI: Front Panel State >> Open
        # "Initialization Macro\n(This is called once, when the VI starts)"
        n137 = local read "Project Folder"() -> (w338:path)
        n138 = call-poly <userlib>:"Valid Path__ogtk.vi"("path"=w338) -> ("valid"=w337:bool)
        n139 = Select(t="Macro: Load Project", s=w337, f="") -> (s? t:f=w334:string)
        n140 = call <vilib>:"Add State(s) to Queue__JKI_lib_State_Machine.vi"("State(s) in Front (\"\")"=w339, "State(s) in (\"\")"=w343, "State(s) at Back (\"\")"=w334) -> ("States Out"=w342:string)  [unwired: 12 in]
      }
      frame "Macro: Load Project" {
        n141 = call <vilib>:"Add State(s) to Queue__JKI_lib_State_Machine.vi"("State(s) in Front (\"\")"="UI: Cursor Set Busy\nProject: Load\nUI: Show First Row of Project Items\nUI: Update Files\nUI: Select All Project Items\nUI: Cursor Set Idle", "State(s) in (\"\")"=w348) -> ("States Out"=w347:string)  [unwired: 13 in]
      }
      frame "Macro: Exit" {
        # "Exit Macro\n(This is called once, when the VI exits)"
        n142 = Unbundle By Name(w355) -> ("Core.Close Panel on Exit?"=w354:bool)
        n143 = Select(t="UI: Front Panel State >> Close", s=w354, f="") -> (s? t:f=w351:string)
        n144 = call <vilib>:"Add State(s) to Queue__JKI_lib_State_Machine.vi"("State(s) in (\"\")"=w351, "State(s) at Back (\"\")"="UI: Uninitialize\nData: Cleanup\nExit") -> ("States Out"=w349:string)  [unwired: 13 in]
        n145 = call <vilib>:"Add State(s) to Queue__JKI_lib_State_Machine.vi"("State(s) in Front (\"\")"=w349, "State(s) in (\"\")"=w358) -> ("States Out"=w357:string)  [unwired: 13 in]
      }
      frame "---------- Project ----------" {
        n146 = call <vilib>:"Add State(s) to Queue__JKI_lib_State_Machine.vi"("State(s) in (\"\")"=w362) -> ("States Out"=w361:string)  [unwired: 14 in]
      }
      frame "Project: Load" {
        n147 = call "Create.vi"("error in (no error)"=w366, "Source Folder"="Project Folder") -> ("error out"=w369:errorcluster, "Session out"=w370:refnum<class "Session.lvclass">)  [unwired: 8 in]
        n148 = local write "Status"("Loading Project" ("Status")) -> ()
        n149 = call "Add Folder Recursively.vi"("error in (no error)"=w369, "Folder"="Project Folder", "Session in"=w370) -> ("error out"=w367:errorcluster, "Session out"=w364:refnum<class "Session.lvclass">)  [unwired: 7 in]
        n150 = Bundle By Name(cluster=w371, "Session"=w364) -> (w365:T7)
        n151 = call <vilib>:"Add State(s) to Queue__JKI_lib_State_Machine.vi"("State(s) in (\"\")"=w373) -> ("States Out"=w372:string)  [unwired: 14 in]
      }
      frame "Project: Refresh" {
        n152 = Unbundle By Name(w376) -> ("Session"=w375:refnum<class "Session.lvclass">)
        n153 = call "Refresh Files Info.vi"("error in (no error)"=w379, "Session in"=w375) -> ("error out"=w378:errorcluster, "Session out"=w377:refnum<class "Session.lvclass">)  [unwired: 8 in]
        n154 = local write "Status"("Reloading Project" ("Status")) -> ()
        n155 = Bundle By Name(cluster=w376, "Session"=w377) -> (w380:T7)
        n156 = call <vilib>:"Add State(s) to Queue__JKI_lib_State_Machine.vi"("State(s) in (\"\")"=w382) -> ("States Out"=w381:string)  [unwired: 14 in]
      }
      frame "Project: Save for Previous" {
        n157 = property on="Files" class="MCListbox (strict)"() -> ("ItemNames"=w393:string[][], "Value"=w395:i32[])  [unwired: 2 in, 2 out]
        n158 = Index Array(array=w393, index (col)=0 ("disabled index (col)")) -> (element=w392:string[])  [unwired: 1 in]
        n159 = Unbundle By Name(w398) -> ("Session"=w389:refnum<class "Session.lvclass">)
        n160 = call-poly <userlib>:"Index Array Elements__ogtk.vi"("indices"=w395, "array"=w392) -> ("elements"=w391:string[])  [unwired: 9 in]
        n161 = String To Path(string=w391) -> (path=w390:path[])
        n162 = call "Write LabVIEW Version.vi"("error in (no error)"=w386, "LabVIEW Version"="LabVIEW Version", "Session in"=w389) -> ("error out"=w387:errorcluster, "Session out"=w388:refnum<class "Session.lvclass">)  [unwired: 7 in]
        n163 = Format Into String(format string="Saving Project Files for LabVIEW %s" ("Status"), "LabVIEW Version") -> (resulting string=w384:string)  [unwired: 2 in, 1 out]
        n164 = call "Save Files for Previous Version.vi"("error in (no error)"=w387, "LabVIEW Files to Convert"=w390, "Session in"=w388) -> ("error out"=w399:errorcluster, "Session out"=w396:refnum<class "Session.lvclass">)  [unwired: 7 in]
        n165 = local write "Status"(w384) -> ()
        n166 = Bundle By Name(cluster=w398, "Session"=w396) -> (w397:T7)
        n167 = call <vilib>:"Add State(s) to Queue__JKI_lib_State_Machine.vi"("State(s) in (\"\")"=w401) -> ("States Out"=w400:string)  [unwired: 14 in]
      }
    }
  }
